vi "Publish Feedback.vi"(8 "error in":errorcluster, 10 "Channel Feedback":T1, 11 "Rig in":refnum<class "Rig.lvclass">) -> (0 "error out":errorcluster, 3 "Rig out":refnum<class "Rig.lvclass">)   [LabVIEW 2026, in "Rig.lvclass"]
doc: "Publishes the given Channel Feedback to the caller as a Channel Feedback Msg. Static, protected. The feedback value is passed in (the rig's Channels field is not read here; see DESIGN_AF_EXECUTOR.md deviation note)."
uses:
  Rig.lvclass
  <vilib>/ActorFramework/Actor/Actor.lvclass/Actor.ctl
  Executor Messages/Channel Feedback Msg/Channel Feedback Msg.lvclass/Channel Feedback Msg.ctl
  <vilib>/ActorFramework/Message Enqueuer/Message Enqueuer.lvclass/Message Enqueuer.ctl
  <vilib>/ActorFramework/Message Enqueuer/Enqueue.vi
  Executor Messages/Channel Feedback Msg/Channel Feedback Msg.lvclass
  <vilib>/ActorFramework/Message Priority Queue/Priority Enqueue.vi
  Rig.lvclass/Rig.ctl
  <vilib>/ActorFramework/Actor/Actor.lvclass
  Typedefs/Channel Value.ctl
  Typedefs/Channel Feedback.ctl
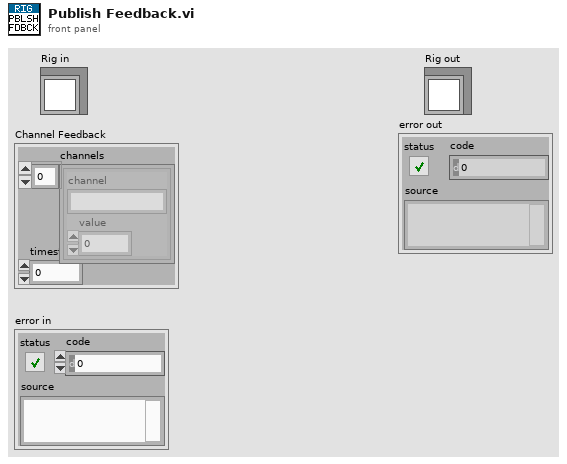
[diagram p1: front panel]
types:
  T1 = typedef "Channel Feedback.ctl" = cluster{"channels":T2[], "timestamp_ms":dbl}
  T2 = typedef "Channel Value.ctl" = cluster{"channel":string, "value":dbl}
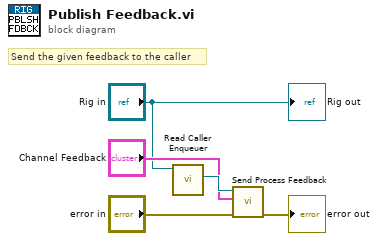
[diagram p0: block diagram]
diagram:
  # "Send the given feedback to the caller"
  n1 = call <vilib>:"Read Caller Enqueuer.vi"("Actor"="Rig in") -> ("Caller Enqueuer"=w5:refnum<class "Message Enqueuer.lvclass">)  [unwired: 10 in]
  n2 = call "Send Process Feedback.vi"("error in (no error)"="error in", "Channel Feedback"="Channel Feedback", "Message Enqueuer"=w5) -> ("error out"=→"error out":errorcluster)  [unwired: 7 in, 1 out]
  "Rig out" <- "Rig in"
